vi "PositionProfileMove.vi"(6 "Immediate?":bool, 7 "Relative?":bool, 8 "error in (no error)":errorcluster, 10 "Array":dbl[](array[numeric]), 11 "SoftmotionAxis in":refnum<class "SoftmotionAxis.lvclass">) -> (0 "error out":errorcluster, 3 "SoftmotionAxis out":refnum<class "SoftmotionAxis.lvclass">)   [LabVIEW 2017, in "SoftmotionAxis.lvclass"]
uses:
  SoftmotionAxis.lvclass
  <resource>/objmgr/nimotion.rc
  Utilities/WordManipulationLibrary.lvlib
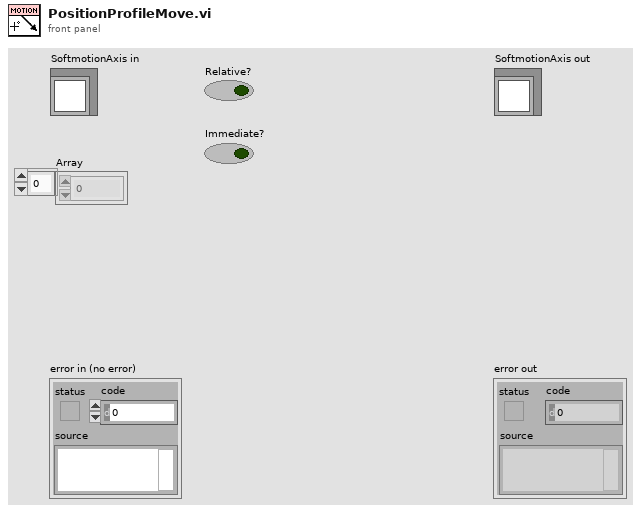
[diagram p1: front panel]
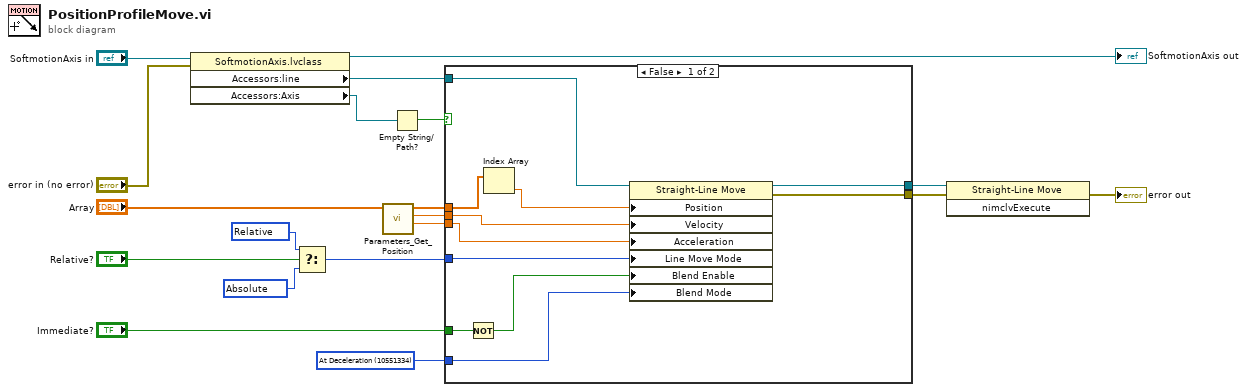
[diagram p0: block diagram]
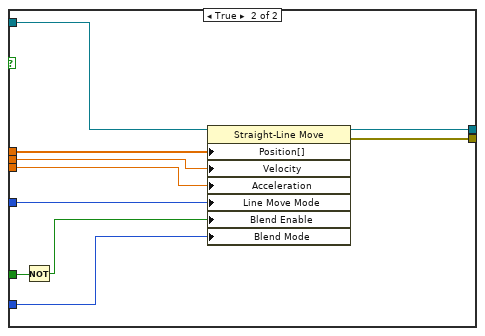
[diagram p2: hidden frame]
diagram:
  w1 = 10551334 items=["At Profile Complete"=10551335, "At Deceleration"=10551334, "After Delay"=10551336] ("Blend Mode")
  w5 = 10551337 items=["Relative"=10551344, "Absolute"=10551337, "Relative To Capture"=10551345, "Velocity"=10551346, "Polyline"=11600101] ("Line Move Mode")
  w4 = 10551344 items=["Relative"=10551344, "Absolute"=10551337, "Relative To Capture"=10551345, "Velocity"=10551346, "Polyline"=11600101] ("Line Move Mode")
  n1 = property class="SoftmotionAxis.lvclass"(reference="SoftmotionAxis in", error in="error in (no error)") -> (reference out=→"SoftmotionAxis out":refnum<class "SoftmotionAxis.lvclass">, "Accessors:line"=w15:refnum<k20>, "Accessors:Axis"=w14:refnum<k21>)  [unwired: 1 out]
  n2 = Select(t=w4, s="Relative?", f=w5) -> (s? t:f=w3:i32)
  n3 = call "Parameters_Get_Position.vi"("Parameters"="Array") -> ("Acceleration"=w10:dbl, "Velocity"=w11:dbl, "Target Position"=w12:dbl[])  [unwired: 7 in, 1 out]
  n4 = Empty String/Path?(string/path=w14) -> (empty?=w13:bool)
  n5 = case shown="False" w13 {
    tunnel: w15 -> [w30 w40]
    tunnel: w12 -> [w29 w39]
    tunnel: w11 -> [w27 w38]
    tunnel: w10 -> [w26 w37]
    tunnel: [w25 w36] -> w8
    tunnel: [w24 w35] -> w7
    tunnel: w3 -> [w23 w34]
    tunnel: "Immediate?" -> [w22 w33]
    tunnel: w1 -> [w20 w31]
    frame False {
      n6 = Not(x=w22) -> (.not. x?=w21:bool)
      n7 = Index Array(array=w29) -> (element=w28:dbl)  [unwired: 1 in]
      n8 = property class="Straight-Line Move"(reference=w30, "Position"=w28, "Velocity"=w27, "Acceleration"=w26, "Line Move Mode"=w23, "Blend Enable"=w21, "Blend Mode"=w20) -> (reference out=w25:refnum<k20>, error out=w24:errorcluster)  [unwired: 1 in]
    }
    frame True {
      n9 = Not(x=w33) -> (.not. x?=w32:bool)
      n10 = property class="Straight-Line Move"(reference=w40, "Position[]"=w39, "Velocity"=w38, "Acceleration"=w37, "Line Move Mode"=w34, "Blend Enable"=w32, "Blend Mode"=w31) -> (reference out=w36:refnum<k20>, error out=w35:errorcluster)  [unwired: 1 in]
    }
  }
  n11 = invoke class="Straight-Line Move" method="nimclvExecute"(reference=w8, error in=w7) -> (error out=→"error out":errorcluster)  [unwired: 1 in, 2 out]
